vi "Get User Interface Information.vi"(8 "error in (no error)":errorcluster, 11 "measurement plugin service in":refnum<class "Measurement Plugin Service.lvclass">) -> (0 "error out":errorcluster, 2 "user interface information":T1[](array[typedef]), 3 "measurement plugin service out":refnum<class "Measurement Plugin Service.lvclass">)   [LabVIEW 2021, in "NI Measurement Plug-In SDK.lvlib" / "Measurement Plugin Service.lvclass"]
doc: "Provides information about the user interfaces supported by the measurement if any. The user interface file can be specified using either a relative or absolute paths. When using a relative path, the path should be relative to the Measurement Logic.vi for the measurement."
uses:
  Measurement Plugin Service.lvclass
  Helpers/TypeDefs/User Interface Information.ctl
  NI Measurement Plug-In SDK.lvlib
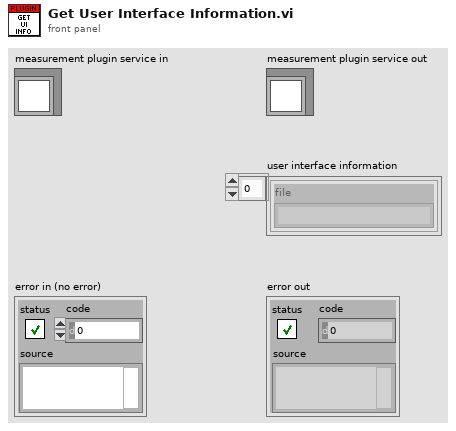
[diagram p1: front panel]
types:
  T1 = typedef "NI Measurement Plug-In SDK.lvlib/User Interface Information.ctl" = cluster{"file":string}
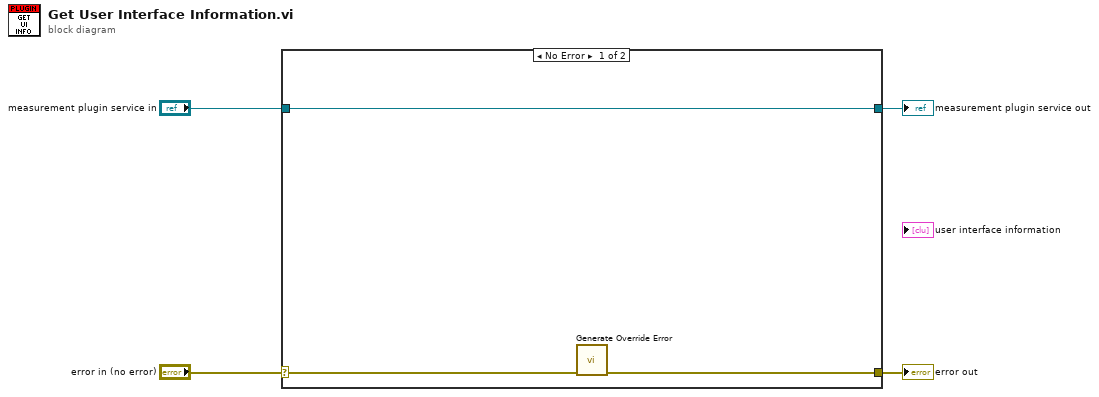
[diagram p0: block diagram]
diagram:
  n1 = case shown="No Error" "error in (no error)" {
    selector: "error in (no error)" -> [w5 w9]
    tunnel: [w6 w9] -> w3
    tunnel: [w7 w8] -> w1
    tunnel: "measurement plugin service in" -> [w7 w8]
    frame No Error {
      n2 = call "Generate Override Error.vi"("error in (no error)"=w5) -> ("error out"=w6:errorcluster)  [unwired: 10 in]
    }
    frame Error {
    }
  }
  "error out" <- w3
  "measurement plugin service out" <- w1
